vi "Set_Output.vi"(8 "error in (no error)":errorcluster, 10 "Output":bool, 11 "object in":refnum<class "DIO_Channel.lvclass">) -> (0 "error out":errorcluster, 3 "object out":refnum<class "DIO_Channel.lvclass">)   [LabVIEW 2021, in "Simulator-Channel.lvlib" / "DIO_Channel.lvclass"]
doc: "Sets the Digital Output"
uses:
  DIO_Channel.lvclass
  C:/Users/averna/Documents/LV Gym DEMO/Factory Pattern/Device Channels/Dependencies/DIO-Channel.lvlibp/Channels/DIO-Channel/DIO_Channel_class/DIO_Channel.lvclass
  DIO_Channel.lvclass/DIO_Channel.ctl
  Panel/DIO_Panel Messages/Set Output Msg/Set Output Msg.lvclass/Set Output Msg.ctl
  <vilib>/ActorFramework/Message Enqueuer/Message Enqueuer.lvclass/Message Enqueuer.ctl
  <vilib>/ActorFramework/Message Enqueuer/Enqueue.vi
  Panel/DIO_Panel Messages/Set Output Msg/Set Output Msg.lvclass
  C:/Program Files/National Instruments/LabVIEW 2021/vi.lib/ActorFramework/Message/Message.lvclass
  Dependencies/DIO-Channel.lvlibp/Channels/DIO-Channel/DIO_Channel_class/Properties/GetDIOConfiguration.vi
  <vilib>/ActorFramework/Message Priority Queue/Priority Enqueue.vi
  Dependencies/DIO-Channel.lvlibp/Channels/DIO-Channel/DIO-Configuration_class/DIO-Configuration.lvclass
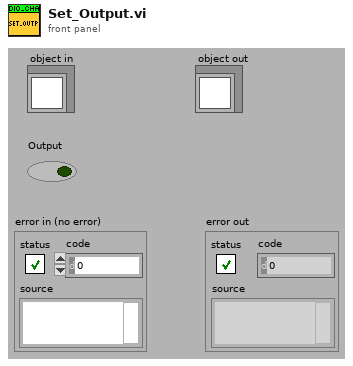
[diagram p1: front panel]
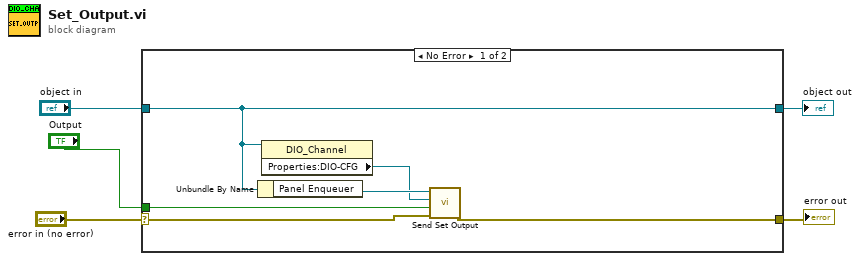
[diagram p0: block diagram]
diagram:
  n1 = case shown="No Error" "error in (no error)" {
    selector: "error in (no error)" -> [w8 w13]
    tunnel: [w7 w13] -> w4
    tunnel: [w9 w12] -> w2
    tunnel: "object in" -> [w9 w12]
    tunnel: "Output" -> [w6 _]
    frame No Error {
      n2 = Unbundle By Name(w9) -> ("Panel Enqueuer"=w11:refnum<class "Message Enqueuer.lvclass">)
      n3 = property class="DIO_Channel"(reference=w9) -> ("Properties:DIO-CFG"=w10:refnum<class "DIO-Configuration.lvclass">)  [unwired: 1 in, 2 out]
      n4 = call "Send Set Output.vi"("error in (no error)"=w8, "Set Output"=w6, "DIO_CFG"=w10, "Message Enqueuer"=w11) -> ("error out"=w7:errorcluster)  [unwired: 6 in, 1 out]
    }
    frame Error {
    }
  }
  "error out" <- w4
  "object out" <- w2
